vi "Get cif_can_writer_nixnet_GetCANStatusResponse.vi"(8 "error in (no error)":errorcluster, 11 "gRPCid":T1) -> (0 "error out":errorcluster, 2 "package_templatemessage":T2, 3 "gRPCid out":T1)   [LabVIEW 2021, in "CanWriterNixnet_server.lvlib"]
uses:
  CanWriterNixnet_server.lvlib
  cif_can_writer_nixnet_GetCANStatusResponse.ctl
  cif_can_writer_nixnet_CommState.ctl
  cif_can_writer_nixnet_LastError.ctl
  <vilib>/gRPC/LabVIEW gRPC Library/Shared/grpcId.ctl
  cif_can_writer_nixnet_GetCANStatusResponse_Flat.ctl
  2ed25e12-861d-4677-8ead-ace2906b2041.vi
  <vilib>/gRPC/LabVIEW gRPC Library/Shared/TranslateGrpcError.vi
  <vilib>/gRPC/LabVIEW gRPC Library/Server API/Server/Get Server DLL Path.vi
  <vilib>/Utility/error.llb/Error Cluster From Error Code.vi
  <vilib>/gRPC/LabVIEW gRPC Library/grpc-lvsupport-release.lvlib
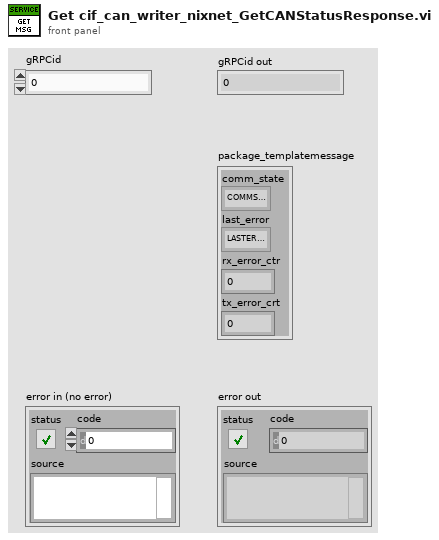
[diagram p1: front panel]
types:
  T1 = typedef "grpc-lvsupport-release.lvlib/grpcId.ctl" = u64
  T2 = typedef "CanWriterNixnet_server.lvlib/cif_can_writer_nixnet_GetCANStatusResponse.ctl" = cluster{"comm_state":T3, "last_error":T4, "rx_error_ctr":u32, "tx_error_crt":u32}
  T3 = typedef "CanWriterNixnet_server.lvlib/cif_can_writer_nixnet_CommState.ctl" = enum32{"COMMSTATE_ERROR_ACTIVE", "COMMSTATE_ERROR_PASSIVE", "COMMSTATE_BUS_OFF"}
  T4 = typedef "CanWriterNixnet_server.lvlib/cif_can_writer_nixnet_LastError.ctl" = enum32{"LASTERROR_NONE", "LASTERROR_STUFF", "LASTERROR_FORM", "LASTERROR_ACK", "LASTERROR_BIT1", "LASTERROR_BIT0", "LASTERROR_CRC", "LASTERROR_UNKNOWN"}
  T5 = typedef "CanWriterNixnet_server.lvlib/cif_can_writer_nixnet_GetCANStatusResponse_Flat.ctl" = cluster{"comm_state":T3, "last_error":T4, "rx_error_ctr":u32, "tx_error_crt":u32}
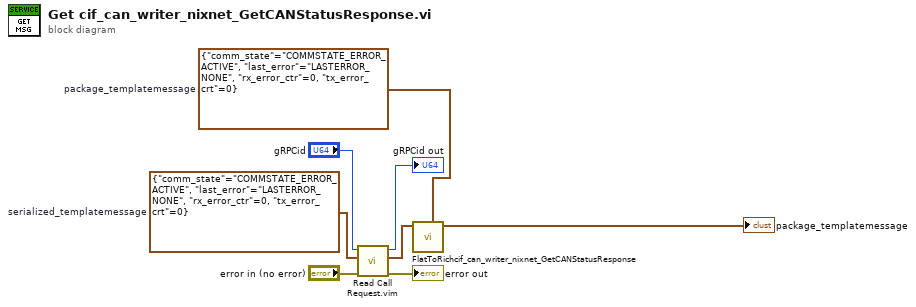
[diagram p0: block diagram]
diagram:
  w6 = T5 {"comm_state"=enum."COMMSTATE_ERROR_ACTIVE", "last_error"=enum."LASTERROR_NONE", "rx_error_ctr"=0, "tx_error_crt"=0}  # serialized_templatemessage
  w5 = T2 {"comm_state"=enum."COMMSTATE_ERROR_ACTIVE", "last_error"=enum."LASTERROR_NONE", "rx_error_ctr"=0, "tx_error_crt"=0}  # package_templatemessage
  n1 = call "Read Call Request.vim"("error in"="error in (no error)", "Request Type"=w6, "gRPCid in"="gRPCid") -> ("error out"=→"error out":errorcluster, "Request Data"=w4:T5, "gRPCid out"=→"gRPCid out":T1)  [unwired: 6 in]
  n2 = call "FlatToRichcif_can_writer_nixnet_GetCANStatusResponse.vi"("OutputClusterType"=w5, "InputCluster"=w4) -> ("OutputCluster"=→"package_templatemessage":T2)  [unwired: 9 in]
